vi "Test MQTT-2.3.1-7.vi"(8 "error in (no error)":errorcluster, 11 "Connection Config":refnum<class "Connection.lvclass">) -> (0 "error out":errorcluster, 3 "Connection Config dup":refnum<class "Connection.lvclass">)   [LabVIEW 2013]
uses:
  <vilib>/LabVIEW Open Source Project/MQTT Connection/MQTT_Connection/Connection/Connection.lvclass
  <vilib>/LabVIEW Open Source Project/MQTT Control Packets/Control Packets/SUBSCRIBE/Topic Subscription -- cluster.ctl
  <vilib>/LabVIEW Open Source Project/MQTT Control Packets/Control Packets/ControlPacket/QualityOfService -- enum.ctl
  <vilib>/addons/_JKI Toolkits/Caraya/classes/Assert/Assert Not Equal Value_Variant.vi
  <vilib>/addons/_JKI Toolkits/Caraya/classes/Test/Test.lvclass
  <vilib>/LabVIEW Open Source Project/MQTT Client/Client class/Client.lvclass
  <vilib>/LabVIEW Open Source Project/MQTT Control Packets/Control Packets/SUBSCRIBE/SUBSCRIBE.lvclass
  <vilib>/LabVIEW Open Source Project/MQTT Control Packets/Control Packets/ControlPacket/ControlPacket.lvclass
  <vilib>/addons/_JKI Toolkits/Caraya/classes/Assert/Assert.lvclass
  <vilib>/LabVIEW Open Source Project/MQTT Connection/MQTT_Base/Base Class/MQTT_Base.lvclass
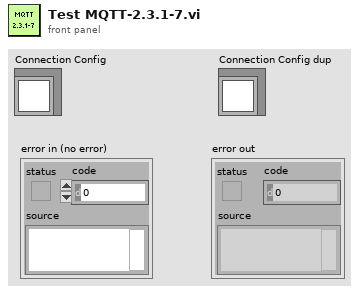
[diagram p1: front panel]
types:
  T1 = typedef "MQTT_Control_Packets.lvlib/SUBSCRIBE.lvclass/Topic Subscription -- cluster.ctl" = cluster{"Topic Filter":string, "QoS":T2}
  T2 = typedef "MQTT_Control_Packets.lvlib/ControlPacket.lvclass/QualityOfService -- enum.ctl" = enum16{"0 (At Most Once)", "1 (At Least Once)", "2 (Exactly Once)"}
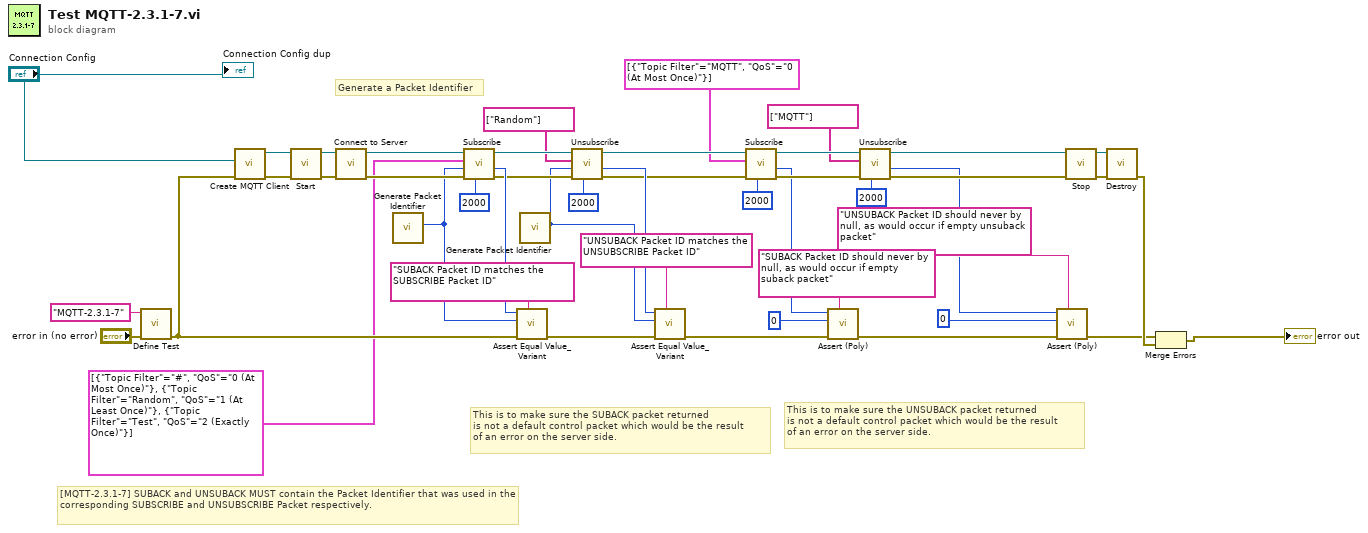
[diagram p0: block diagram]
diagram:
  # "This is to make sure the UNSUBACK packet returned\nis not a default control packet which would be the result\nof an error on the server side."
  # "This is to make sure the SUBACK packet returned\nis not a default control packet which would be the result\nof an error on the server side."
  # "Generate a Packet Identifier"
  # "[MQTT-2.3.1-7] SUBACK and UNSUBACK MUST contain the Packet Identifier that was used in the corresponding SUBSCRIBE and UNSUBSCRIBE Packet respectively."
  n1 = call <vilib>:"Define Test.vi"("error in (no error)"="error in (no error)", "Label (VI Title)"="MQTT-2.3.1-7") -> ("error out"=w33:errorcluster)  [unwired: 9 in]
  n2 = call <vilib>:"Create MQTT Client.vi"("error in (no error)"=w33, "Connection Configuration"="Connection Config") -> ("error out"=w35:errorcluster, "Client out"=w36:refnum<class "Client.lvclass">)  [unwired: 8 in]
  n3 = call <vilib>:"Start.vi"("error in (no error)"=w35, "MQTT_Base in"=w36) -> ("error out"=w42:errorcluster, "MQTT_Base out"=w43:refnum<class "Client.lvclass">)  [unwired: 7 in, 1 out]
  n4 = call <vilib>:"Connect to Server.vi"("error in (no error)"=w42, "Client in"=w43) -> ("error out"=w38:errorcluster, "Client out"=w39:refnum<class "Client.lvclass">)  [unwired: 6 in, 2 out]
  n5 = call <vilib>:"Generate Packet Identifier.vi"() -> ("Packet Identifier"=w29:u16)  [unwired: 11 in]
  n6 = call <vilib>:"Subscribe.vi"("timeout (1000 ms)"=2000, "error in (no error)"=w38, "Packet ID (empty: Generate new)"=w29, "Topic Subscriptions"=T1[] [{"Topic Filter"="#", "QoS"=enum."0 (At Most Once)"}, {"Topic Filter"="Random", "QoS"=enum."1 (At Least Once)"}, {"Topic Filter"="Test", "QoS"=enum."2 (Exactly Once)"}], "MQTT_Base in"=w39) -> ("error out"=w27:errorcluster, "SUBACK Packet ID"=w30:u16, "MQTT_Base out"=w28:refnum<class "Client.lvclass">)  [unwired: 3 in, 1 out]
  n7 = call <vilib>:"Assert Equal Value_Variant.vi"("Label"="SUBACK Packet ID matches the SUBSCRIBE Packet ID", "error in (no error)"=w33, "Y"=w29, "X"=w30) -> ("error out"=w24:errorcluster)  [unwired: 7 in]
  n8 = call <vilib>:"Generate Packet Identifier.vi"() -> ("Packet Identifier"=w21:u16)  [unwired: 11 in]
  n9 = call <vilib>:"Unsubscribe.vi"("timeout (1000 ms)"=2000, "error in (no error)"=w27, "Packet ID (empty: Generate new)"=w21, "Topics"=string[] ["Random"], "MQTT_Base in"=w28) -> ("error out"=w19:errorcluster, "UNSUBACK Packet ID"=w23:u16, "MQTT_Base out"=w20:refnum<class "Client.lvclass">)  [unwired: 4 in]
  n10 = call <vilib>:"Assert Equal Value_Variant.vi"("Label"="UNSUBACK Packet ID matches the UNSUBSCRIBE Packet ID", "error in (no error)"=w24, "Y"=w21, "X"=w23) -> ("error out"=w10:errorcluster)  [unwired: 7 in]
  n11 = call <vilib>:"Subscribe.vi"("timeout (1000 ms)"=2000, "error in (no error)"=w19, "Topic Subscriptions"=T1[] [{"Topic Filter"="MQTT", "QoS"=enum."0 (At Most Once)"}], "MQTT_Base in"=w20) -> ("error out"=w15:errorcluster, "SUBACK Packet ID"=w9:u16, "MQTT_Base out"=w16:refnum<class "Client.lvclass">)  [unwired: 4 in, 1 out]
  n12 = call-poly <vilib>:"Assert (Poly).vi"("Label"="SUBACK Packet ID should never by null, as would occur if empty suback packet", "error in (no error)"=w10, "Y"=u16 0 ("SUBACK Packet ID"), "X"=w9) -> ("error out"=w6:errorcluster)  [unwired: 7 in]
  n13 = call <vilib>:"Unsubscribe.vi"("timeout (1000 ms)"=2000, "error in (no error)"=w15, "Topics"=string[] ["MQTT"], "MQTT_Base in"=w16) -> ("error out"=w14:errorcluster, "UNSUBACK Packet ID"=w3:u16, "MQTT_Base out"=w13:refnum<class "Client.lvclass">)  [unwired: 5 in]
  n14 = call-poly <vilib>:"Assert (Poly).vi"("Label"="UNSUBACK Packet ID should never by null, as would occur if empty unsuback packet", "error in (no error)"=w6, "Y"=u16 0 ("SUBACK Packet ID"), "X"=w3) -> ("error out"=w5:errorcluster)  [unwired: 7 in]
  n15 = call <vilib>:"Stop.vi"("error in (no error)"=w14, "MQTT_Base in"=w13) -> ("error out"=w40:errorcluster, "MQTT_Base out"=w41:refnum<class "Client.lvclass">)  [unwired: 7 in, 1 out]
  n16 = call <vilib>:"Destroy.vi"("error in (no error)"=w40, "MQTT_Base in"=w41) -> ("error out"=w31:errorcluster)  [unwired: 8 in, 1 out]
  n17 = Merge Errors(w5, w31) -> (→"error out":errorcluster)
  "Connection Config dup" <- "Connection Config"
